vi "PracticaCayetanoVI.vi"() -> ()   [LabVIEW 2025]
uses:
  <vilib>/Instr/_visa.llb/VISA Configure Serial Port (Instr).vi
panel:
  in  "Send Hysteresis":bool
  in  "W OFF":dbl
  in  "W ON":dbl
  in  "Cluster":T1={"Speed or Position"=0, "Kp"=0.497, "Ki"=6.531, "Kd"=0.00232} {"Speed or Position" items=["Speed", "Position"]}
  out "Last Read":string
  out "Waveform Chart 2":dbl(graph)
  out "Boolean":bool
  out "Waveform Chart":cluster{dbl, dbl}(graph)
  in  "Send Gains":bool
  in  "REFERENCE":dbl=75.0
  in  "MODE":enum16{"Wave", "Speed", "Position"}(ring)
  out "read buffer":string
  in  "baud rate":u32=115200
  in  "VISA resource name":refnum<visa-resource-name>
  in  "stop":bool
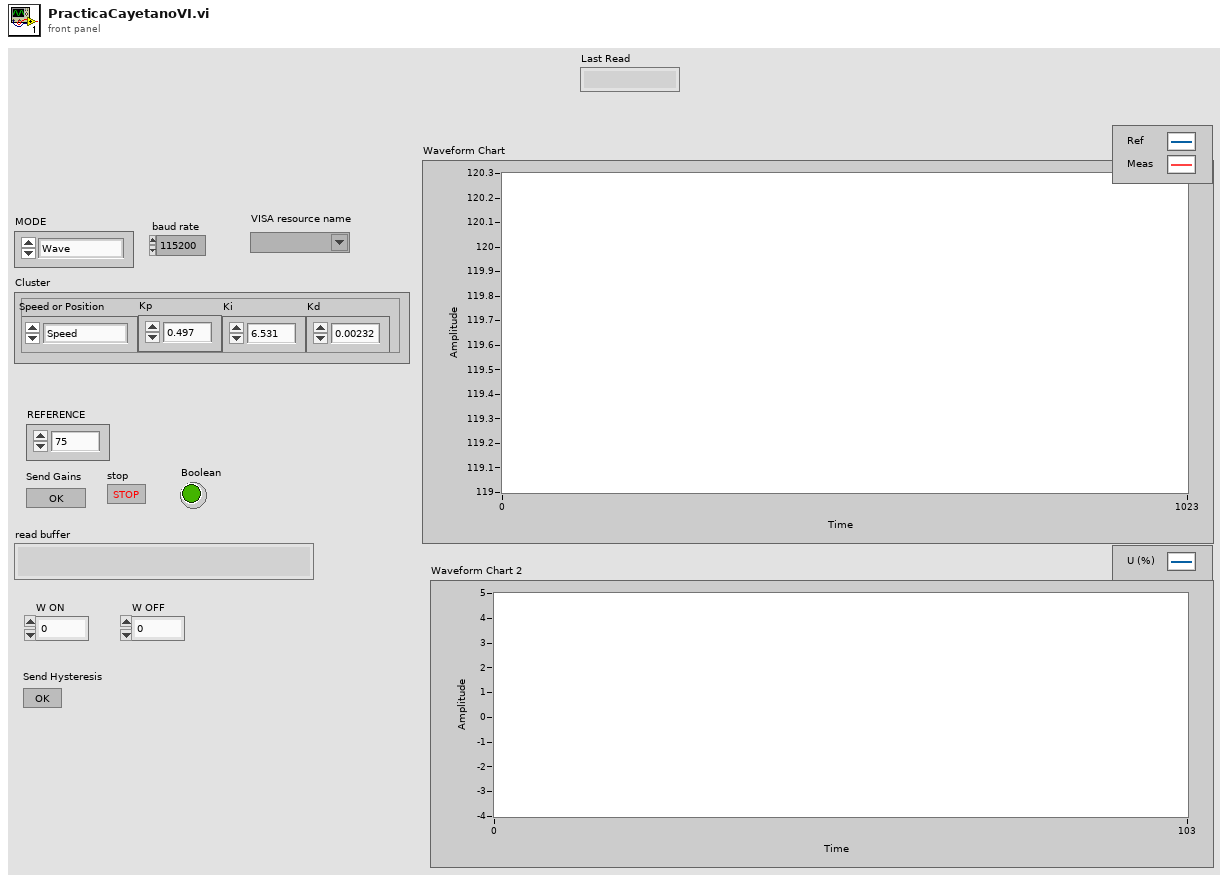
[diagram p1: front panel]
types:
  T1 = cluster{"Speed or Position":u16, "Kp":dbl, "Ki":dbl, "Kd":dbl}
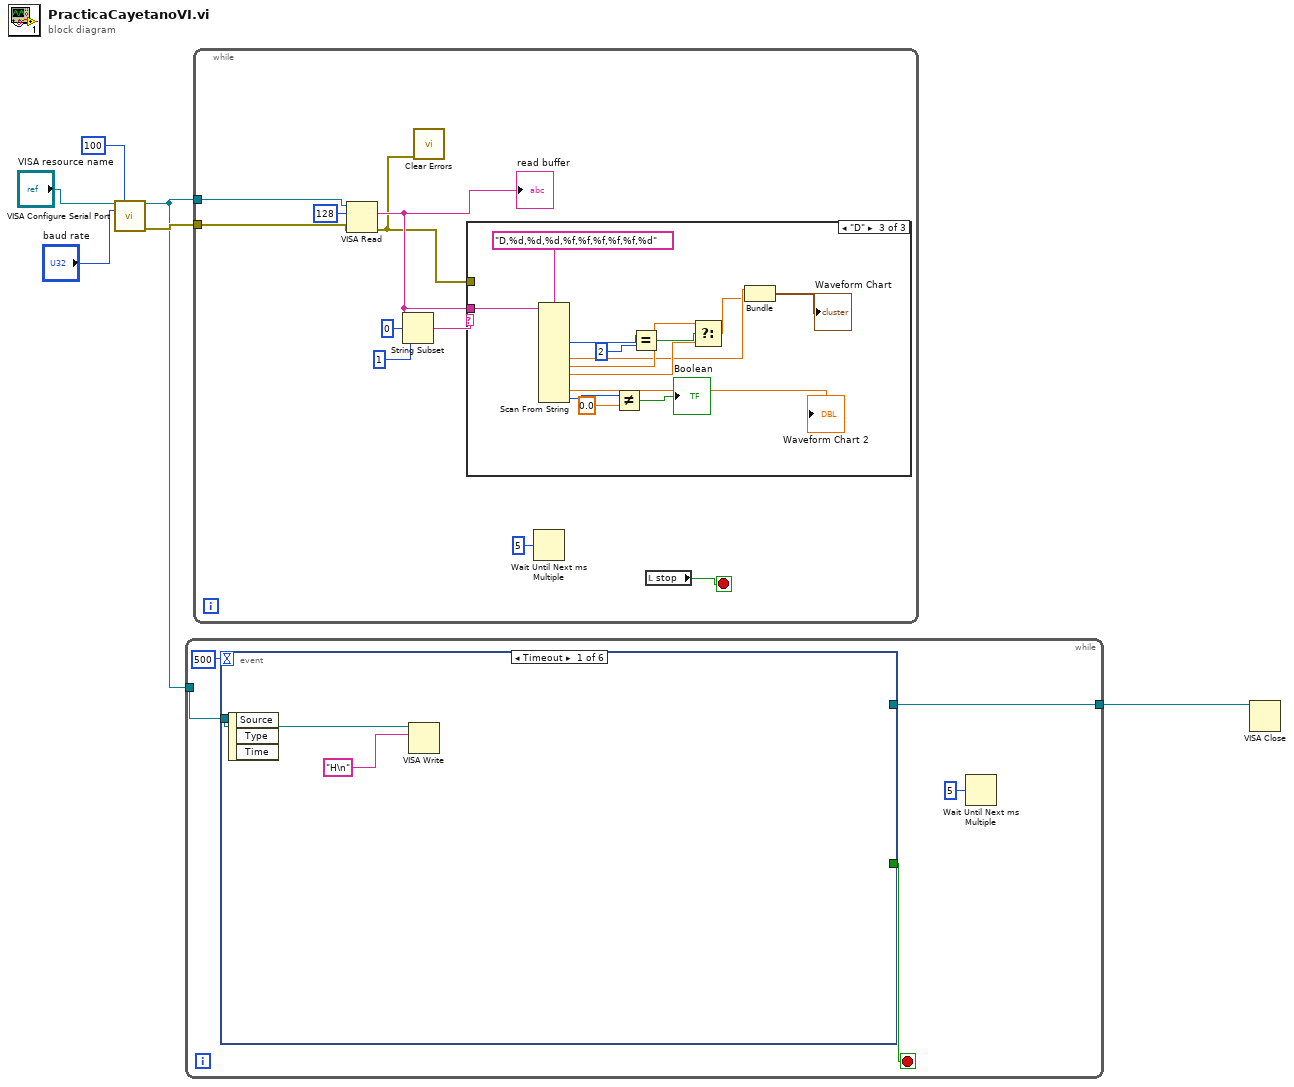
[diagram p0: block diagram]
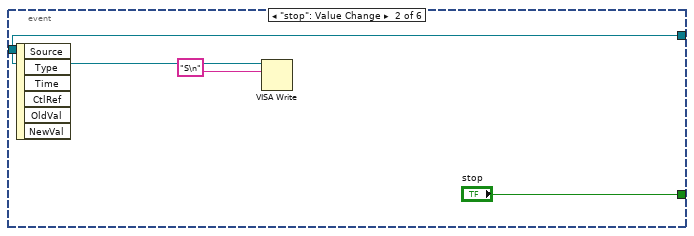
[diagram p2: hidden frame]
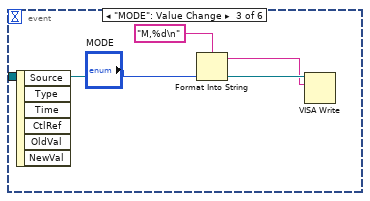
[diagram p3: hidden frame]
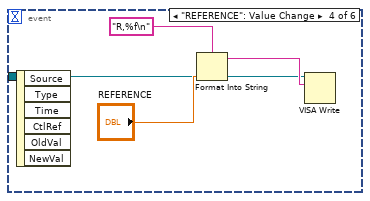
[diagram p4: hidden frame]
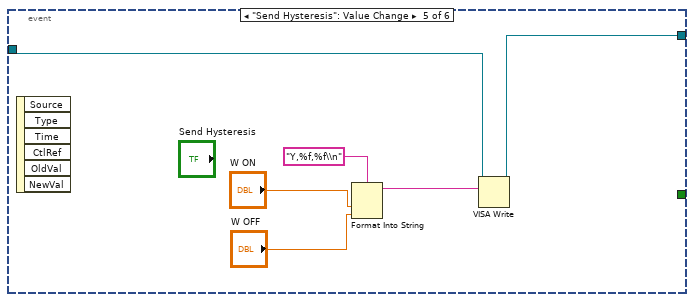
[diagram p5: hidden frame]
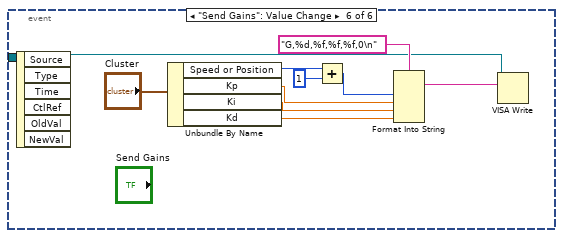
[diagram p6: hidden frame]
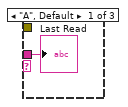
[diagram p7: hidden frame]
diagram:
  n1 = call-poly "VISA Configure Serial Port"("VISA resource name"="VISA resource name", "timeout (10sec)"=u32 100, "baud rate (9600)"="baud rate") -> ("VISA resource name out"=w3:refnum<visa-resource-name>, "error out"=w4:errorcluster)  [unwired: 11 in]
  n2 = while {
    tunnel: w3 -> [w11]
    tunnel: [w8] -> w2
    stop <- w9 stop-if-true
    n3 = event shown="[0] Timeout" {
      selector: _ -> [_ _ _ _ _ _]
      dyn-events: _ -> [_ _ _ _ _ _]
      timeout: 500 -> [_ _ _ _ _ _]
      tunnel: w11 -> [w13 w14 w19 w22 w26 w32]
      tunnel: [_ "stop" _ _ _ _] -> w9
      tunnel: [_ w14 _ _ w25 _] -> w8
      event Timeout {
        n4 = event-data() -> ()  [unwired: 1 in, 3 out]
        n5 = VISA Write(VISA resource name=w13, write buffer="H\n") -> ()  [unwired: 1 in, 3 out]
      }
      event "stop": Value Change {
        n6 = event-data() -> ()  [unwired: 1 in, 6 out]
        n7 = VISA Write(VISA resource name=w14, write buffer="S\n") -> ()  [unwired: 1 in, 3 out]
      }
      event "MODE": Value Change {
        n8 = event-data() -> ()  [unwired: 1 in, 6 out]
        n9 = Format Into String(format string="M,%d\n" ("initial string"), "MODE") -> (resulting string=w18:string)  [unwired: 2 in, 1 out]
        n10 = VISA Write(VISA resource name=w19, write buffer=w18) -> ()  [unwired: 1 in, 3 out]
      }
      event "REFERENCE": Value Change {
        n11 = event-data() -> ()  [unwired: 1 in, 6 out]
        n12 = Format Into String(format string="R,%f\n" ("initial string"), "REFERENCE") -> (resulting string=w24:string)  [unwired: 2 in, 1 out]
        n13 = VISA Write(VISA resource name=w22, write buffer=w24) -> ()  [unwired: 1 in, 3 out]
      }
      event "Send Hysteresis": Value Change {
        n14 = event-data() -> ()  [unwired: 1 in, 6 out]
        n15 = Format Into String(format string="Y,%f,%f\\n", "W ON", "W OFF") -> (resulting string=w27:string)  [unwired: 2 in, 1 out]
        n16 = VISA Write(VISA resource name=w26, write buffer=w27) -> (VISA resource name out=w25:refnum<visa-resource-name>)  [unwired: 1 in, 2 out]
      }
      event "Send Gains": Value Change {
        n17 = event-data() -> ()  [unwired: 1 in, 6 out]
        n18 = Unbundle By Name("Cluster") -> ("Speed or Position"=w39:u16, "Kp"=w36:dbl, "Ki"=w35:dbl, "Kd"=w34:dbl)
        n19 = Add(x=w39, y=u16 1) -> (x+y=w37:u16)
        n20 = Format Into String(format string="G,%d,%f,%f,%f,0\n", w37, w36, w35, w34) -> (resulting string=w31:string)  [unwired: 2 in, 1 out]
        n21 = VISA Write(VISA resource name=w32, write buffer=w31) -> ()  [unwired: 1 in, 3 out]
      }
    }
    n22 = Wait Until Next ms Multiple(millisecond multiple=u32 5) -> ()  [unwired: 1 out]
  }
  n23 = while {
    tunnel: w3 -> [w50]
    tunnel: w4 -> [w48]
    stop <- w43 stop-if-true
    n24 = VISA Read(VISA resource name=w50, byte count=u32 128, error in (no error)=w48) -> (read buffer=w44:string, error out=w42:errorcluster)  [unwired: 2 out]
    "read buffer" <- w44
    n25 = String Subset(string=w44, offset (0)=0, length (rest)=1 ("length (rest)")) -> (substring=w45:string)
    n26 = call <vilib>:"Clear Errors.vi"("error in (no error)"=w42) -> ()  [unwired: 5 in, 2 out]
    n27 = case shown="\"D\"" w45 {
      tunnel: w42 -> [_ _ _]
      tunnel: w44 -> [w51 _ w64]
      frame "A", Default {
        "Last Read" <- w51
      }
      frame "N" {
      }
      frame "D" {
        n28 = Scan From String(format string="D,%d,%d,%d,%f,%f,%f,%f,%f,%d", input string=w64) -> (output 2=w60:i32, output 4=w55:dbl, output 5=w57:dbl, output 6=w56:dbl, output 8=→"Waveform Chart 2":dbl, output 9=w62:i32)  [unwired: 14 in, 3 out]
        n29 = Not Equal?(x=w62, y=0.0) -> (x != y?=→"Boolean":bool)
        n30 = Equal?(x=w60, y=2) -> (x = y?=w58:bool)
        n31 = Select(t=w57, s=w58, f=w56) -> (s? t:f=w54:dbl)
        n32 = Bundle(w55, w54) -> (→"Waveform Chart":cluster{dbl, dbl})  [unwired: 1 in]
      }
    }
    n33 = Wait Until Next ms Multiple(millisecond multiple=u32 5) -> ()  [unwired: 1 out]
    n34 = local read "stop"() -> (w43:bool)
  }
  n35 = VISA Close(VISA resource name=w2) -> ()  [unwired: 1 in, 1 out]
